vi "Test Round Trip.vi"(8 "error in (no error)":errorcluster) -> (0 "error out":errorcluster)   [LabVIEW 2019, in "RemoteControl.ZMQ.Tests.lvclass"]
uses:
  RemoteControl.ZMQ.Tests.lvclass
  C:/Program Files/National Instruments/LabVIEW 2019/user.lib/LevyLab/RemoteControl/RemoteControl/RemoteControl.lvclass
  <userlib>/LevyLab/RemoteControl/RemoteControl/RemoteControl.lvclass/RemoteControl.ctl
  <vilib>/numeric/Random Number (Range) U64.vi
  ea5dac89-44c8-4270-b814-2c06dabdc587.vi
  <vilib>/numeric/sub_Random U32.vi
  ea5dac89-44c8-4270-b814-2c06dabdc587.vi/8a413093-aa11-4f93-94f1-5b9fe02facac.vi
  ea5dac89-44c8-4270-b814-2c06dabdc587.vi/b885af2a-e049-452f-b1a7-e5e1b9c14209.vi
  <vilib>/addons/_JKI Toolkits/Caraya/classes/Assert/Assert Not Error.vi
  <vilib>/Utility/Data Type/Get Type Information.vi
  <vilib>/JDP Science/JSONtext/JSON text to Variant.vi
  <vilib>/addons/_JKI Toolkits/Caraya/classes/Assert/Assert Equal Value_Variant.vi
  <vilib>/JDP Science/JSONtext/LVClass Serializer/JSONtext LVClass Serializer.lvclass
  <userlib>/LevyLab/RemoteControl/RemoteControl/RemoteControl.lvclass
  <vilib>/addons/_JKI Toolkits/Caraya/classes/Assert/Assert.lvclass
  <vilib>/addons/_JKI Toolkits/Caraya/classes/Test/Test.lvclass
panel:
  out "client error out":errorcluster
  out "server error out":errorcluster
  out "Commands from server":string[](array[string])
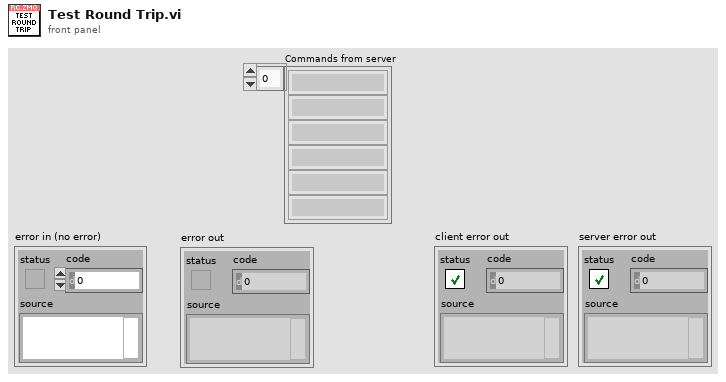
[diagram p1: front panel]
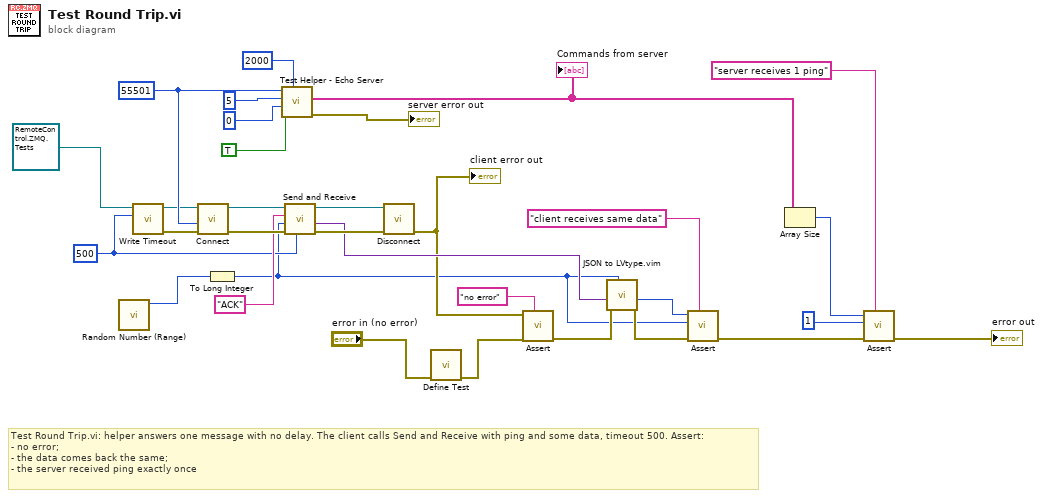
[diagram p0: block diagram]
diagram:
  w6 = 500 ("timeout in ms (100)")
  w28 = u16 55501 ("Port")
  # "Test Round Trip.vi: helper answers one message with no delay. The client calls Send and Receive with ping and some data, timeout 500. Assert:\n- no error;\n- the data comes back the same;\n- the server received ping exactly once"
  n1 = call-poly <vilib>:"Random Number (Range).vi"() -> ("number"=w16:u64)  [unwired: 11 in]
  n2 = call <userlib>:"Write Timeout.vi"("timeout (ms) [500]"=w6, "RemoteControl in"=refnum<class "RemoteControl.ZMQ.Tests.lvclass"> refnum ("RemoteControl.ZMQ.Tests.lvclass")) -> ("error out"=w15:errorcluster, "RemoteControl out"=w14:refnum<class "RemoteControl.ZMQ.Tests.lvclass">)  [unwired: 8 in]
  n3 = call <userlib>:"Connect.vi"("error in (no error)"=w15, "Port"=w28, "RemoteControl in"=w14) -> ("error out"=w30:errorcluster, "RemoteControl out"=w32:refnum<class "RemoteControl.ZMQ.Tests.lvclass">)  [unwired: 7 in]
  n4 = To Long Integer(number=w16) -> (32bit integer=w2:i32)
  n5 = call "Test Helper - Echo Server.vi"("idle timout"=u32 2000, "Answer?"=TRUE, "reply delay (ms)"=u32 0, "number of messages"=5, "port"=w28) -> ("error out"=→"server error out":errorcluster, "Commands"=w23:string[])  [unwired: 5 in]
  "Commands from server" <- w23
  n6 = call <userlib>:"Send and Receive.vi"("timeout (ms) [500]"=w6, "error in (no error)"=w30, "Data"=w2, "Command"="ACK", "RemoteControl in"=w32) -> ("error out"=w29:errorcluster, "Data out"=w12:variant, "RemoteControl out"=w31:refnum<class "RemoteControl.ZMQ.Tests.lvclass">)  [unwired: 3 in, 1 out]
  n7 = call <userlib>:"Disconnect.vi"("error in (no error)"=w29, "RemoteControl in"=w31) -> ("error out"=w3:errorcluster)  [unwired: 8 in, 1 out]
  "client error out" <- w3
  n8 = call <vilib>:"Define Test.vi"("error in (no error)"="error in (no error)") -> ("error out"=w8:errorcluster)  [unwired: 9 in, 1 out]
  n9 = call-poly <vilib>:"Assert.vi"("Label"="no error", "error in (no error)"=w8, "Not Error?"=w3) -> ("error out"=w10:errorcluster)  [unwired: 7 in, 1 out]
  n10 = call "JSON to LVtype.vim"("type"=w2, "error in (no error)"=w10, "JSON Data in"=w12) -> ("error out"=w9:errorcluster, "Data out"=w11:i32)  [unwired: 7 in]
  n11 = call-poly <vilib>:"Assert.vi"("Label"="client receives same data", "error in (no error)"=w9, "Actual"=w2, "Expected"=w11) -> ("error out"=w21:errorcluster)  [unwired: 6 in, 1 out]
  n12 = Array Size(array=w23) -> (size(s)=w22:i32)
  n13 = call-poly <vilib>:"Assert.vi"("Label"="server receives 1 ping", "error in (no error)"=w21, "Actual"=1 ("size(s)"), "Expected"=w22) -> ("error out"=→"error out":errorcluster)  [unwired: 6 in, 1 out]
